vi "Get Unbundler.vi"(8 "error in (no error)":errorcluster, 10 "Label":string, 11 "Owner VI in":refnum<vi>) -> (0 "error out":errorcluster, 1 "Found ?":bool, 2 "Unbundler Refnum":refnum<vi>, 3 "Owner VI out":refnum<vi>)   [LabVIEW 2019, in "gRPC Template Creation Utility.lvlib"]
uses:
  gRPC Template Creation Utility.lvlib
  <vilib>/Utility/traverseref.llb/TRef TravTarget.ctl
  <vilib>/Utility/traverseref.llb/VI Scripting - Traverse.lvlib
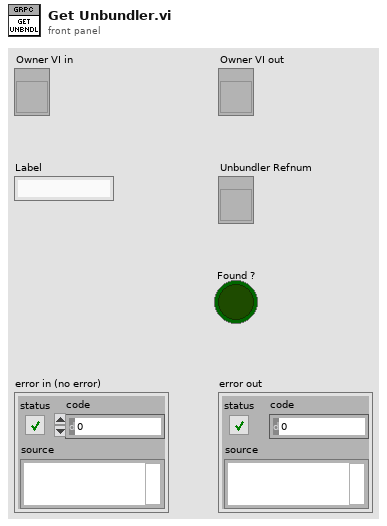
[diagram p1: front panel]
types:
  T1 = typedef "TRef TravTarget.ctl" = enum16{"FP", "BD", "Other"}
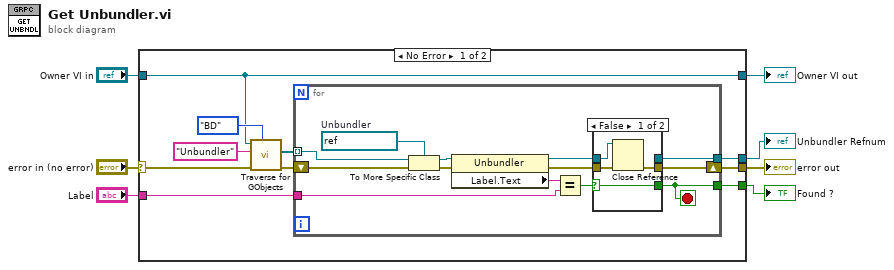
[diagram p0: block diagram]
diagram:
  n1 = case shown="No Error" "error in (no error)" {
    selector: "error in (no error)" -> [w11 w38]
    tunnel: "Label" -> [w17 _]
    tunnel: "Owner VI in" -> [w10 w39]
    tunnel: [w8 w38] -> w5
    tunnel: [w12 _] -> w1
    tunnel: [w10 w39] -> w3
    tunnel: [w9 _] -> w2
    frame No Error {
      n2 = call <vilib>:"Traverse for GObjects.vi"("Traverse Target"=TRef_TravTarget."BD", "error in (no error)"=w11, "Class Name"="Unbundler", "VI Refnum"=w10) -> ("error out"=w13:errorcluster, "References"=w16:refnum<vi>[])  [unwired: 4 in, 2 out]
      n3 = for {
        tunnel: w16 -> [w30] mode=indexing
        tunnel: w17 -> [w26]
        tunnel: [w23] -> w12
        tunnel: [w21] -> w9
        shift-right: [w18] -> w8
        shift-left: w13 -> [w29]
        stop <- w21 stop-if-true
        w19 = refnum<vi> refnum  # Unbundler
        n4 = To More Specific Class(target class=w19, reference=w30, error in=w29) -> (specific class reference=w28:refnum<vi>, error out=w20:errorcluster)
        n5 = property class="Unbundler"(reference=w28, error in=w20) -> (reference out=w24:refnum<vi>, error out=w22:errorcluster, "Label.Text"=w27:string)
        n6 = Equal?(x=w27, y=w26) -> (x = y?=w25:bool)
        n7 = case shown="False" w25 {
          selector: w25 -> [w31 w35]
          tunnel: w24 -> [w34 w37]
          tunnel: [_ w37] -> w23
          tunnel: [w31 w35] -> w21
          tunnel: w22 -> [w33 w36]
          tunnel: [w32 w36] -> w18
          frame False {
            n8 = Close Reference(reference=w34, error in (no error)=w33) -> (error out=w32:errorcluster)
          }
          frame True {
          }
        }
      }
    }
    frame Error {
    }
  }
  "error out" <- w5
  "Owner VI out" <- w3
  "Found ?" <- w2
  "Unbundler Refnum" <- w1
